vi "CSE ISP - Save text file.vi"(5 "ena prompt":bool, 6 "pattern":string, 7 "prompt":string, 8 "error in":errorcluster, 9 "default name":string, 10 "data":string, 11 "path":path) -> (0 "error out":errorcluster, 1 "cancelled":bool, 3 "path out":path)   [LabVIEW 2021]
doc: "::: CalcExpress Toolkit :::\nCopyright (c) 2000-2026 Konstantin Shifershteyn. All rights reserved."
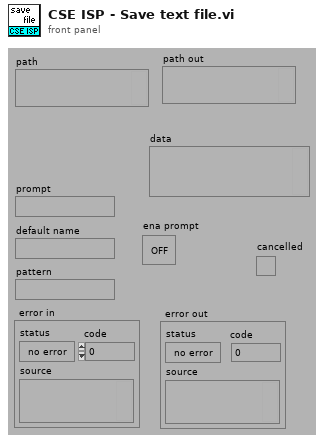
[diagram p1: front panel]
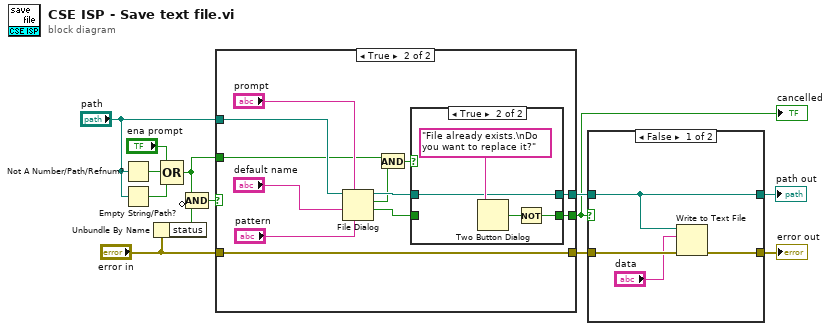
[diagram p0: block diagram]
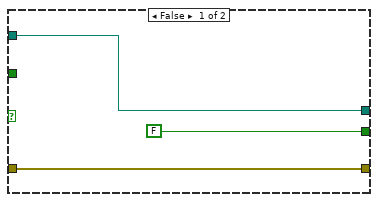
[diagram p3: hidden frame]
diagram:
  n1 = Not A Number/Path/Refnum?(number/path/refnum="path") -> (NaN/Path/Refnum?=w8:bool)
  n2 = Empty String/Path?(string/path="path") -> (empty?=w7:bool)
  n3 = Unbundle By Name("error in") -> ("status"=w11:bool)
  n4 = Compound Arithmetic op=OR("ena prompt", w8, w7) -> (w1:bool)
  n5 = Compound Arithmetic op=AND(w1, invert w11) -> (w9:bool)
  n6 = case shown="True" w9 {
    tunnel: [w15 w22] -> w5
    tunnel: [w16 w21] -> w6
    tunnel: "error in" -> [w16 w21]
    tunnel: "path" -> [w15 w18]
    tunnel: [FALSE ("cancelled") w24] -> w3
    tunnel: w1 -> [_ w17]
    frame False {
    }
    frame True {
      n7 = File Dialog(6:"pattern", 7:"prompt", 9:"default name", 11:w18) -> (1:w25:bool, 2:w19:bool, 3:w23:path)  [unwired: 3 in, 1 out]
      n8 = And(x=w17, y=w19) -> (x .and. y?=w20:bool)
      n9 = case shown="True" w20 {
        tunnel: [w30 w31] -> w24
        tunnel: w25 -> [w30 _]
        tunnel: w23 -> [w29 w32]
        tunnel: [w29 w32] -> w22
        frame False {
        }
        frame True {
          n10 = Two Button Dialog(message="File already exists.\nDo you want to replace it?") -> (T button?=w33:bool)  [unwired: 2 in]
          n11 = Not(x=w33) -> (.not. x?=w31:bool)
        }
      }
    }
  }
  "cancelled" <- w3
  n12 = case shown="False" w3 {
    tunnel: [w37 w40] -> w13
    tunnel: w6 -> [w38 w40]
    tunnel: w5 -> [w36 w39]
    tunnel: [w36 w39] -> w4
    frame False {
      n13 = Write to Text File(file (use dialog)=w36, text="data", error in=w38) -> (error out=w37:errorcluster)  [unwired: 1 in, 2 out]
    }
    frame True {
    }
  }
  "error out" <- w13
  "path out" <- w4
